vi "model_in_out_port.vi"() -> ()   [LabVIEW 2020]
uses:
  <vilib>/Model Interface Toolkit/Get Outport Paths.vi
  <vilib>/Model Interface Toolkit/Get Inport Paths.vi
  <vilib>/Model Interface Toolkit/Model Interface Toolkit.lvclass
panel:
  out "Model Period (s)":dbl
  out "outports":string[](array[string])
  out "路径":path
  out "Inports":string[](array[string])
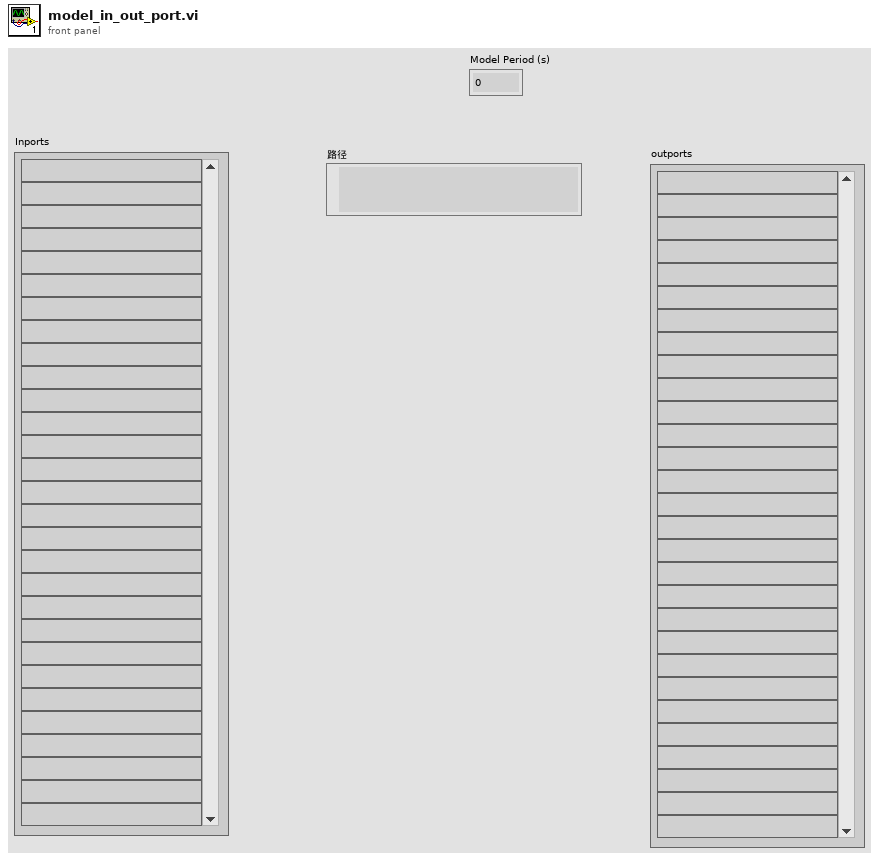
[diagram p1: front panel]
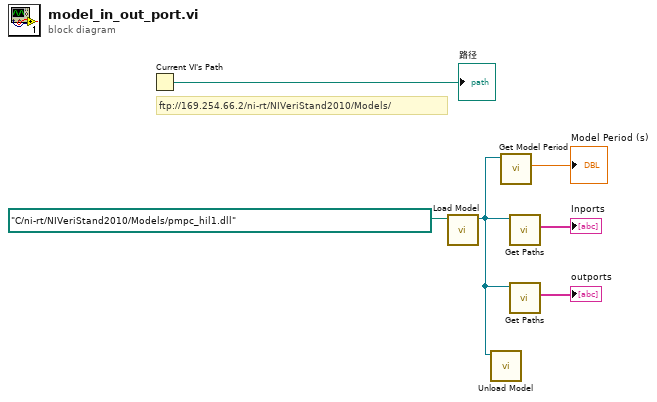
[diagram p0: block diagram]
diagram:
  # "ftp://169.254.66.2/ni-rt/NIVeriStand2010/Models/"
  n1 = Current VI's Path() -> (path=→"路径":path)
  n2 = call <vilib>:"Load Model.vi"("Model Path"=path "C:/ni-rt/NIVeriStand2010/Models/pmpc_hil1.dll") -> ("Model out"=w2:refnum<class "Model Interface Toolkit.lvclass">)  [unwired: 9 in, 1 out]
  n3 = call <vilib>:"Unload Model.vi"("Model in"=w2) -> ()  [unwired: 10 in, 1 out]
  n4 = call <vilib>:"Get Model Period.vi"("Model in"=w2) -> ("Model Period (s)"=→"Model Period (s)":dbl)  [unwired: 8 in, 2 out]
  n5 = call-poly <vilib>:"Get Paths.vi"("Model in"=w2) -> ("Inport Paths"=→"Inports":string[])  [unwired: 8 in, 2 out]
  n6 = call-poly <vilib>:"Get Paths.vi"("Model in"=w2) -> ("Outport Paths"=→"outports":string[])  [unwired: 8 in, 2 out]
